vi "Read Key File.vi"(7 "Key Type":T1, 8 "Error In":errorcluster, 11 "Key File":path) -> (0 "Error Out":errorcluster, 3 "Key Data":string)   [LabVIEW 2017, in "Tests.lvlib"]
uses:
  Tests.lvlib
  SSH Key Types.ctl
  <vilib>/Utility/sysdir.llb/Get System Directory.vi
  <vilib>/Utility/file.llb/Is Path and Not Empty.vi
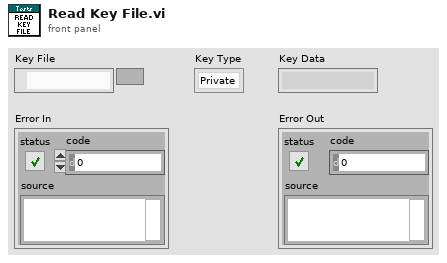
[diagram p1: front panel]
types:
  T1 = typedef "Tests.lvlib/SSH Key Types.ctl" = enum16{"Private", "Public"}
  T2 = enum16{"open", "replace", "create", "open or create", "replace or create", "replace or create with confirmation"}
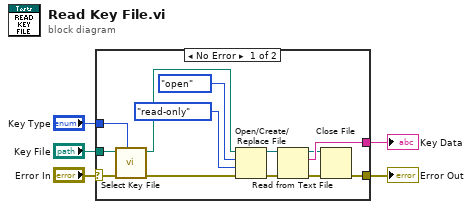
[diagram p0: block diagram]
diagram:
  n1 = case shown="No Error" "Error In" {
    selector: "Error In" -> [w7 w19]
    tunnel: [w18 w19] -> w5
    tunnel: "Key File" -> [w17 _]
    tunnel: [w14 _] -> w3
    tunnel: "Key Type" -> [w6 _]
    frame No Error {
      n2 = call "Select Key File.vi"("Key Type"=w6, "Error In"=w7, "Key File In"=w17) -> ("Error Out"=w15:errorcluster, "Key File Out"=w16:path)  [unwired: 7 in]
      n3 = Open/Create/Replace File(file path (use dialog)=w16, error in=w15, operation (0:open)=T2."open", access (0:read/write)=enum16{"read/write", "read-only", "write-only"}."read-only") -> (refnum out=w10:refnum<file>, error out=w11:errorcluster)  [unwired: 2 in, 1 out]
      n4 = Read from Text File(file (use dialog)=w10, error in=w11) -> (refnum out=w13:refnum<file>, text=w14:string, error out=w12:errorcluster)  [unwired: 2 in, 1 out]
      n5 = Close File(refnum=w13, error in=w12) -> (error out=w18:errorcluster)  [unwired: 1 out]
    }
    frame Error {
    }
  }
  "Error Out" <- w5
  "Key Data" <- w3
